vi "FuncVI-viAbort.vi"(5 "InstanceRef":T2, 9 "arg list":T1[](array[typedef]) {"num" format="%.2f"}) -> (0 "error out":bool, 3 "result":T1 {"num" format="%.2f"})   [LabVIEW 2021]
doc: "::: CalcExpress Toolkit :::\nCopyright (c) 2000-2026 Konstantin Shifershteyn. All rights reserved."
uses:
  cetypes.llb/CalcExpress Function Argument Info.ctl
  cetypes.llb/CalcExpress Instance RefNum.ctl
panel:
  in  "max arg num":i32=2
  in  "min arg num":i32=1
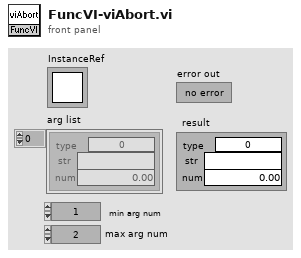
[diagram p1: front panel]
types:
  T1 = typedef "CalcExpress Function Argument Info.ctl" = cluster{"type":u32, "str":string, "num":dbl}
  T2 = typedef "CalcExpress Instance RefNum.ctl" = refnum<k1>
  T3 = enum32{"String", "DBL Number", "identifier", "1D Array of DBL", "2D Array of DBL", "CDB Number", "1D Array of CDB", "2D Array of CDB", "1D Array of String", "2D Array of String", "Unknown data type"}
  T4 = cluster{"index":i32, "data type":enum32{"String", "DBL Number", "identifier", "1D Array of DBL", "2D Array of DBL", "CDB Number", "1D Array of CDB", "2D Array of CDB", "1D Array of String", "2D Array of String", "Unknown data type"}, "default num":dbl, "default str":string}[]
  T5 = cluster{"use this constant to specify a predefined type":enum32{"String", "DBL Number", "identifier", "1D Array of DBL", "2D Array of DBL", "CDB Number", "1D Array of CDB", "2D Array of CDB", "1D Array of String", "2D Array of String", "Unknown data type"}, string, "code":i32}
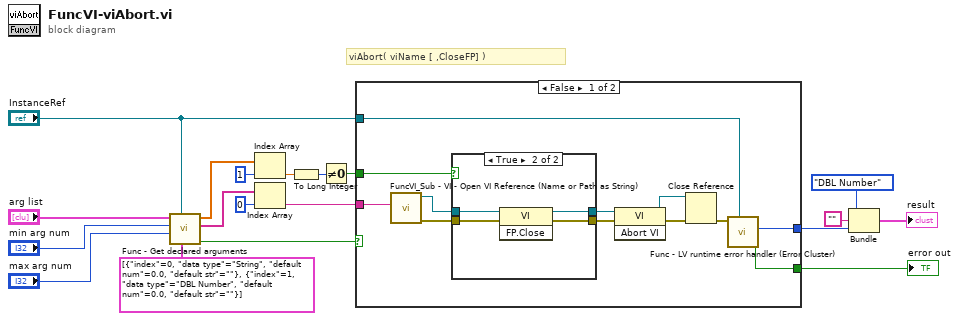
[diagram p0: block diagram]
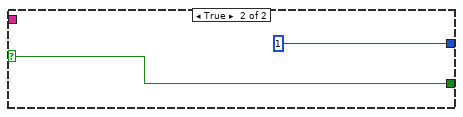
[diagram p3: hidden frame]
diagram:
  # "viAbort( viName [ ,CloseFP] )"
  n1 = call "Func - Get declared arguments.vi"("arg descriptors"=T4 [{"index"=0, "data type"=enum."String", "default num"=0.0, "default str"=""}, {"index"=1, "data type"=enum."DBL Number", "default num"=0.0, "default str"=""}] ("args descriptors"), "InstanceRef"="InstanceRef", "max arg num"="max arg num", "min arg num"="min arg num", "arg list"="arg list") -> ("error out"=w2:bool, "str list"=w12:string[], "num list"=w13:dbl[])  [unwired: 3 in, 1 out]
  n2 = Index Array(array=w13, index=1) -> (element=w10:dbl)
  n3 = Index Array(array=w12, index=0) -> (element=w1:string)
  n4 = To Long Integer(number=w10) -> (32bit integer=w11:i32)
  n5 = Not Equal To 0?(x=w11) -> (x != 0?=w9:bool)
  n6 = case shown="False" w2 {
    selector: w2 -> [_ w39]
    tunnel: w1 -> [w31 _]
    tunnel: w9 -> [w28 _]
    tunnel: [w20 w39] -> w7
    tunnel: "InstanceRef" -> [w22 _]
    tunnel: [w21 1 ("code")] -> w4
    frame False {
      n7 = call "FuncVI_Sub - VI - Open VI Reference (Name or Path as String).vi"("VI name or path"=w31) -> ("error out"=w30:errorcluster, "VI Refnum"=w29:refnum<vi>)  [unwired: 9 in]
      n8 = case shown="True" w28 {
        tunnel: w30 -> [w32 w35]
        tunnel: w29 -> [w33 w37]
        tunnel: [w33 w36] -> w27
        tunnel: [w32 w34] -> w26
        frame False {
        }
        frame True {
          n9 = invoke class="VI" method="FP.Close"(reference=w37, error in=w35) -> (reference out=w36:refnum<vi>, error out=w34:errorcluster)  [unwired: 1 in, 1 out]
        }
      }
      n10 = invoke class="VI" method="Abort VI"(reference=w27, error in=w26) -> (reference out=w24:refnum<vi>, error out=w25:errorcluster)  [unwired: 1 in, 1 out]
      n11 = Close Reference(reference=w24, error in (no error)=w25) -> (error out=w23:errorcluster)
      n12 = call "Func - LV runtime error handler (Error Cluster).vi"("InstanceRef"=w22, "LabVIEW error"=w23) -> ("error out"=w20:bool, "LV error code"=w21:i32)  [unwired: 4 in, 2 out]
    }
    frame True {
    }
  }
  "error out" <- w7
  n13 = Bundle("use this constant to specify a predefined type"=T3."DBL Number", "", "code"=w4) -> (→"result":T5)  [unwired: 1 in]
